vi "InitializeSolenoid.vi"() -> (0 "error out":T1)   [LabVIEW 2014]
uses:
  ErrorOut.ctl
  <vilib>/Rock Robotics/WPI/Solenoid/WPI_SolenoidOpenDouble.vi
  <vilib>/Rock Robotics/WPI/Solenoid/WPI_SolenoidSetEnum.vi
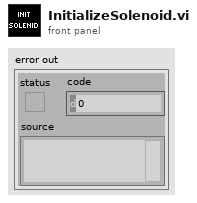
[diagram p1: front panel]
types:
  T1 = typedef "ErrorOut.ctl" = errorcluster
  T2 = typedef "WPI_SolenoidDevRef.ctl" = cluster{"DevStatus":errorcluster, "Pneumatics Control Module":u8, "Forward Solenoid Channel":T3, "Reverse Solenoid Channel":T3}
  T3 = typedef "WPI_SolenoidChannel.ctl" = enum8{"Solenoid 0", "Solenoid 1", "Solenoid 2", "Solenoid 3", "Solenoid 4", "Solenoid 5", "Solenoid 6", "Solenoid 7", "Invalid"}
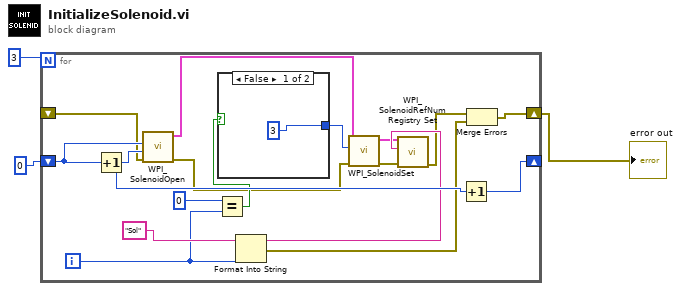
[diagram p0: block diagram]
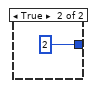
[diagram p2: hidden frame]
diagram:
  n1 = for {
    N: 3 -> [_]
    shift-right: [w18] -> _
    shift-left: 0 -> [w19]
    shift-right: [w5] -> w1
    shift-left: _ -> [w4]
    i -> [w12]
    n2 = Increment(x=w19) -> (x+1=w20:i32)
    n3 = call-poly <vilib>:"WPI_SolenoidOpen.vi"("error in (no error)"=w4, "Reverse Solenoid Channel"=w20, "Forward Solenoid Channel"=w19) -> ("error out"=w9:errorcluster, "SolenoidDevRef"=w8:T2)  [unwired: 7 in]
    n4 = Equal?(x=0, y=w12) -> (x = y?=w11:bool)
    n5 = case shown="False" w11 {
      tunnel: [3 2] -> w10
      frame False {
      }
      frame True {
      }
    }
    n6 = Format Into String(initial string="Sol", w12) -> (resulting string=w16:string, error out=w6:errorcluster)  [unwired: 2 in]
    n7 = call-poly <vilib>:"WPI_SolenoidSet.vi"("error in (no error)"=w9, "Value"=w10, "SolenoidDevRef"=w8) -> ("error out"=w15:errorcluster, "SolenoidDevRef"=w14:T2)  [unwired: 7 in]
    n8 = call <vilib>:"WPI_SolenoidRefNum Registry Set.vi"("error in (no error)"=w15, "refnum name"=w16, "SolenoidDevRef"=w14) -> ("error out"=w7:errorcluster)  [unwired: 7 in, 1 out]
    n9 = Increment(x=w20) -> (x+1=w18:i32)
    n10 = Merge Errors(w7, w6) -> (w5:errorcluster)
  }
  "error out" <- w1
